vi "init.vi"(8 "error in":errorcluster, 10 "TBM module configuration in":refnum<class "TBM module configuration.lvclass">, 11 "fixed channel runtime in":refnum<class "DAQmx Watchdog runtime.lvclass">) -> (0 "error out":errorcluster, 1 "data allocations":T1, 2 "execution settings":T4, 3 "fixed channel runtime out":refnum<class "DAQmx Watchdog runtime.lvclass">)   [LabVIEW 2014, in "DAQmx Watchdog runtime.lvclass"]
doc: "Provides an interface for initializing a module at runtime. While this interface performs no operations, a child should provide an override which may open any necessary references or sessions, allocate necessary memory, and perform any final configuration validataion before providing the full configuration <b>execution data</b> to the calling process."
uses:
  DAQmx Watchdog runtime.lvclass
  <vilib>/NI/Tag Bus Module Framework/module configuration/TBM module configuration.lvclass
  <vilib>/NI/Tag Bus Module Framework/runtime/execution settings.ctl
  <vilib>/NI/Tag Bus Module Framework/channel/data tables.ctl
  <vilib>/NI/Tag Bus/dictionary/data dictionary.lvclass
  <vilib>/NI/Tag Bus/dictionary table pair.ctl
  <vilib>/NI/Tag Bus/table/data table.ctl
  configuration/DAQmx Watchdog configuration.lvclass
  DAQmx Watchdog runtime.lvclass/DAQmx Watchdog runtime.ctl
  <vilib>/DAQmx/configure/task.llb/DAQmx Configure Watchdog Expiration States (Analog Output).vi
  <vilib>/DAQmx/configure/task.llb/DAQmx Configure Watchdog Expiration States (Counter Output).vi
  <vilib>/DAQmx/configure/task.llb/DAQmx Configure Watchdog Expiration States (Digital Output).vi
  <vilib>/NI/DCAF/Tag Editor Core/control module/runtime/control module runtime.lvclass
  <resource>/objmgr/daqmx.rc
  <vilib>/NI/Tag Bus Module Framework/runtime/TBM module execution interface.lvclass
  <vilib>/NI/Tag Bus Module Framework/channel/TBM channel.lvclass
  <vilib>/NI/Tag Bus/tag bus.lvlib
  <vilib>/NI/Tag Bus/table/data table.lvlib
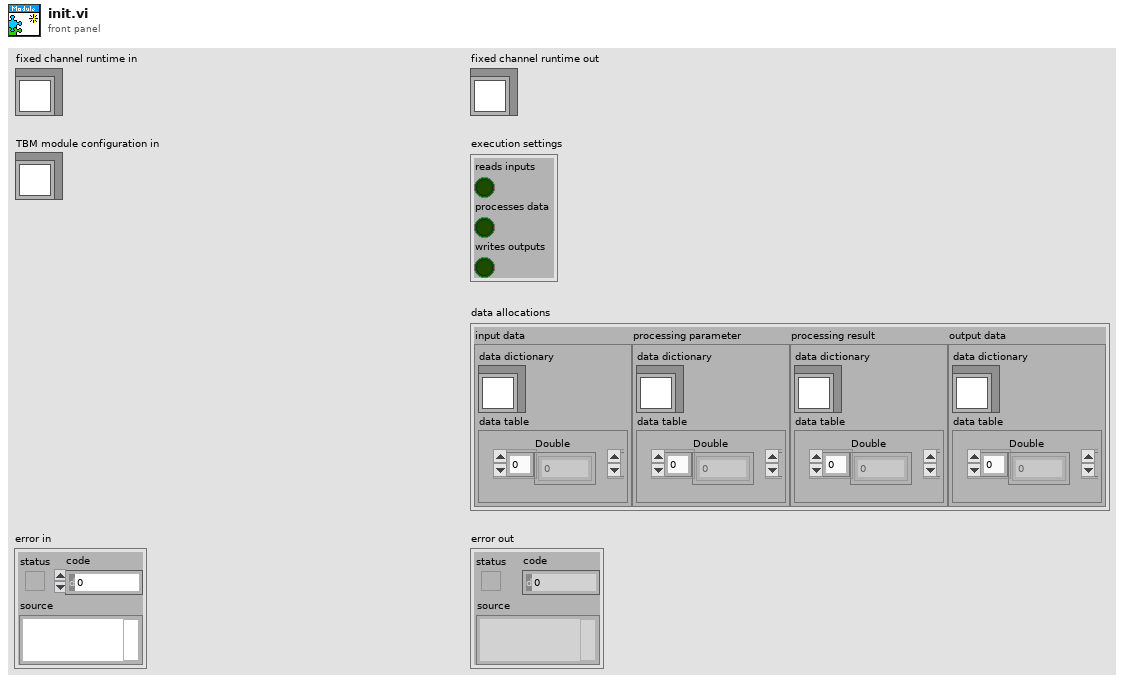
[diagram p1: front panel]
types:
  T1 = typedef "TBM channel.lvclass/data tables.ctl" = cluster{"input data":T2, "processing parameter":T2, "processing result":T2, "output data":T2}
  T2 = typedef "tag bus.lvlib/dictionary table pair.ctl" = cluster{"data dictionary":refnum<class "data dictionary.lvclass">, "data table":T3}
  T3 = typedef "tag bus.lvlib/data table.lvlib/data table.ctl" = cluster{"Double":dbl[], "Single":sgl[], "I64":i64[], "I32":i32[], "I16":i16[], "I8":i8[], "U64":u64[], "U32":u32[], "U16":u16[], "U8":u8[], "Boolean":bool[], "String":string[], "Array of Double":cluster{"DBL Array":dbl[]}[], "Array of Single":cluster{"SGL Array":sgl[]}[], "Array of I64":cluster{"I64 Array":i64[]}[], "Array of I32":cluster{"I32 Array":i32[]}[], "Array of I16":cluster{"I16 Array":i16[]}[], "Array of I8":cluster{"I8 Array":i8[]}[], "Array of U64":cluster{"U64 Array":u64[]}[], "Array of U32":cluster{"U32 Array":u32[]}[], "Array of U16":cluster{"U16 Array":u16[]}[], "Array of U8":cluster{"U8 Array":u8[]}[], "Array of Boolean":cluster{"Boolean Array":bool[]}[], "Array of String":cluster{"String Array":string[]}[]}
  T4 = typedef "TBM module execution interface.lvclass/execution settings.ctl" = cluster{"reads inputs":bool, "processes data":bool, "writes outputs":bool}
  T5 = cluster{"physical channel":tag, "expiration state":dbl, "output type":i32}[]
  T6 = cluster{"physical channel(s)":tag, "expiration state":i32}[]
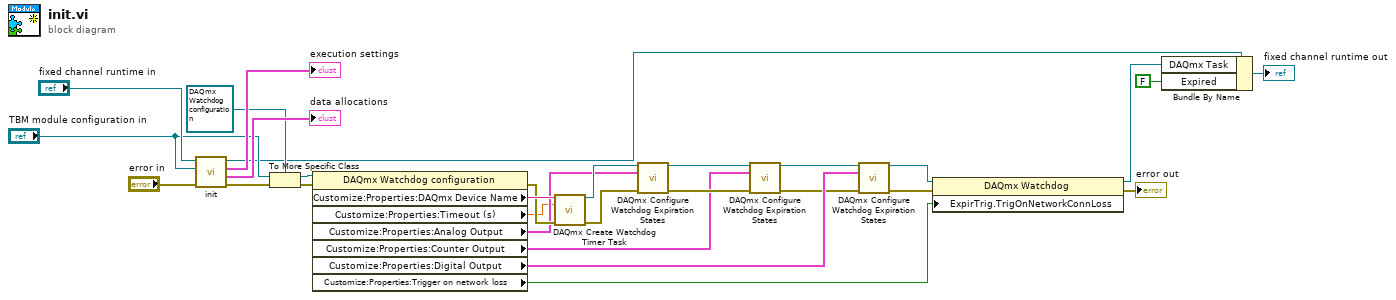
[diagram p0: block diagram]
diagram:
  n1 = call-parent "init.vi"("error in"="error in", "TBM module configuration in"="TBM module configuration in", "fixed channel runtime in"="fixed channel runtime in") -> ("error out"=w20:errorcluster, "data allocations"=→"data allocations":T1, "execution settings"=→"execution settings":T4, "fixed channel runtime out"=w5:refnum<class "DAQmx Watchdog runtime.lvclass">)  [unwired: 5 in]
  n2 = To More Specific Class(target class=refnum<class "DAQmx Watchdog configuration.lvclass"> refnum, reference="TBM module configuration in", error in=w20) -> (specific class reference=w23:refnum<class "DAQmx Watchdog configuration.lvclass">, error out=w24:errorcluster)
  n3 = property class="DAQmx Watchdog configuration"(reference=w23, error in=w24) -> (error out=w21:errorcluster, "Customize:Properties:DAQmx Device Name"=w22:tag, "Customize:Properties:Timeout (s)"=w13:dbl, "Customize:Properties:Analog Output"=w17:T5, "Customize:Properties:Counter Output"=w14:T6, "Customize:Properties:Digital Output"=w11:T6, "Customize:Properties:Trigger on network loss"=w7:bool)  [unwired: 1 out]
  n4 = call <vilib>:"DAQmx Create Watchdog Timer Task.vi"("device in"=w22, "timeout"=w13, "error in"=w21) -> ("task out"=w19:refnum<k21>, "error out"=w18:errorcluster)  [unwired: 11 in]
  n5 = call-poly <vilib>:"DAQmx Configure Watchdog Expiration States.vi"("task in"=w19, "expiration states"=w17, "error in"=w18) -> ("task out"=w15:refnum<k21>, "error out"=w16:errorcluster)  [unwired: 11 in]
  n6 = call-poly <vilib>:"DAQmx Configure Watchdog Expiration States.vi"("task in"=w15, "expiration states"=w14, "error in"=w16) -> ("task out"=w12:refnum<k21>, "error out"=w10:errorcluster)  [unwired: 11 in]
  n7 = call-poly <vilib>:"DAQmx Configure Watchdog Expiration States.vi"("task in"=w12, "expiration states"=w11, "error in"=w10) -> ("task out"=w9:refnum<k21>, "error out"=w8:errorcluster)  [unwired: 11 in]
  n8 = property class="DAQmx Watchdog"(reference=w9, error in=w8, "ExpirTrig.TrigOnNetworkConnLoss"=w7) -> (reference out=w3:refnum<k21>, error out=→"error out":errorcluster)
  n9 = Bundle By Name(cluster=w5, "DAQmx Task"=w3, "Expired"=FALSE) -> (→"fixed channel runtime out":refnum<class "DAQmx Watchdog runtime.lvclass">)
